vi "Get Backup.vi"(7 "output file path":path=path "", 8 "error in (no error)":errorcluster, 9 "to":timestamp format="%<%x>T", 10 "from":timestamp format="%<%x>T", 11 "eLab in":refnum<class "PL eLabFTW Client.lvclass">) -> (0 "error out":errorcluster, 2 "data":string, 3 "eLab out":refnum<class "PL eLabFTW Client.lvclass">)   [LabVIEW 2015, in "PL eLabFTW Client.lvclass"]
doc: "Saves backup with the experiments for the specified time period to the specified path. The backup is ordered by users and contains only the experiments that changed in the specified time period."
uses:
  PL eLabFTW Client.lvclass
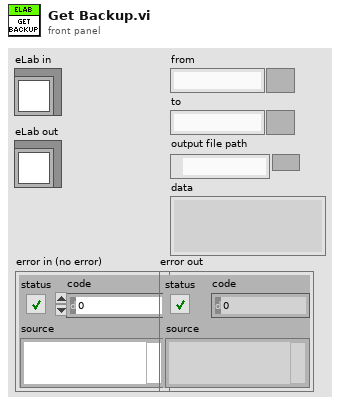
[diagram p1: front panel]
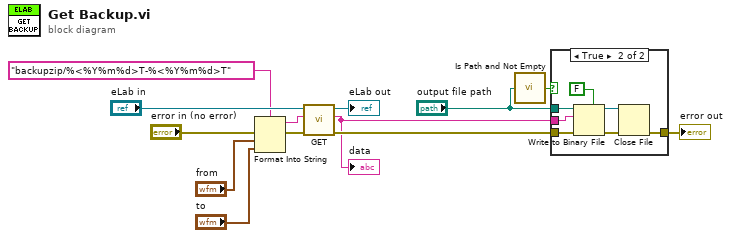
[diagram p0: block diagram]
diagram:
  n1 = Format Into String(format string="backupzip/%<%Y%m%d>T-%<%Y%m%d>T", error in="error in (no error)", "from", "to") -> (resulting string=w11:string, error out=w10:errorcluster)  [unwired: 1 in]
  n2 = call "GET.vi"("error in (no error)"=w10, "relative URL"=w11, "eLab in"="eLab in") -> ("error out"=w3:errorcluster, "response body"=w2:string, "eLab out"=→"eLab out":refnum<class "PL eLabFTW Client.lvclass">)  [unwired: 6 in]
  "data" <- w2
  n3 = call <vilib>:"Is Path and Not Empty.vi"("path"="output file path") -> ("Is Path and Not Empty?"=w4:bool)  [unwired: 4 in]
  n4 = case shown="True" w4 {
    tunnel: w3 -> [w14 w21]
    tunnel: [w14 w17] -> w1
    tunnel: "output file path" -> [_ w20]
    tunnel: w2 -> [_ w15]
    frame False {
    }
    frame True {
      n5 = Write to Binary File(file (use dialog)=w20, data=w15, error in=w21, 5:FALSE ("prepend array or string size? (T)")) -> (refnum out=w18:refnum<file>, error out=w19:errorcluster)  [unwired: 2 in, 1 out]
      n6 = Close File(refnum=w18, error in=w19) -> (error out=w17:errorcluster)  [unwired: 1 out]
    }
  }
  "error out" <- w1
